vi "Copy.vi"(8 "error in":errorcluster, 9 "Target Folder":path, 10 "Source":path, 11 "File Manager in":refnum<class "File Manager.lvclass">) -> (0 "error out":errorcluster, 2 "New Path":path, 3 "File Manager out":refnum<class "File Manager.lvclass">)   [LabVIEW 2026, in "File Manager.lvclass"]
doc: "This VI copies the specified source to the target directory. If the target already exists it will be overwritten."
uses:
  File Manager.lvclass
  File Manager.lvclass/File Manager.ctl
  Interfaces/ILogger/ILogger Messages/Log Msg/Log Msg.lvclass/Log Msg.ctl
  <vilib>/ActorFramework/Message Enqueuer/Message Enqueuer.lvclass/Message Enqueuer.ctl
  <vilib>/ActorFramework/Message Enqueuer/Enqueue.vi
  Interfaces/ILogger/ILogger Messages/Log Msg/Log Msg.lvclass
  <userlib>/_OpenG.lib/file/file.llb/Strip Path Extension - Path__ogtk.vi
  <vilib>/ActorFramework/Message Priority Queue/Priority Enqueue.vi
  <userlib>/_OpenG.lib/file/file.llb/openg_file.lvlib
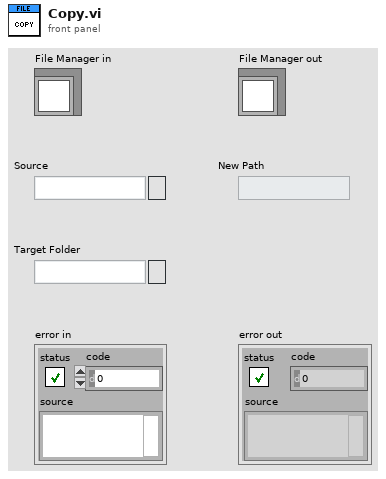
[diagram p1: front panel]
types:
  T1 = typedef "Log Entry--cluster.ctl" = cluster{"Time":timestamp, "Message":string}
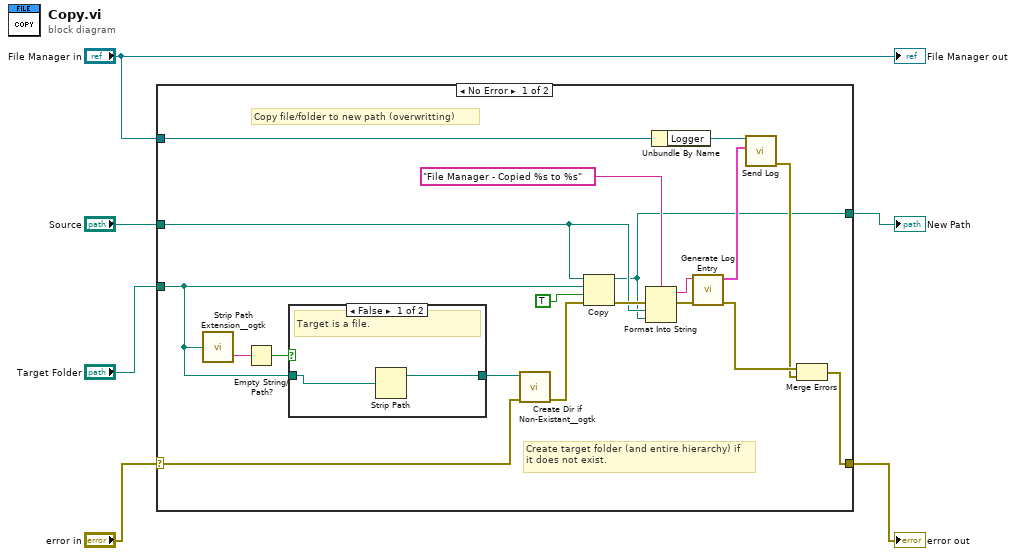
[diagram p0: block diagram]
diagram:
  n1 = case shown="No Error" "error in" {
    selector: "error in" -> [w8 w29]
    tunnel: [w25 w29] -> w6
    tunnel: "File Manager in" -> [w20 _]
    tunnel: "Source" -> [w14 _]
    tunnel: [w13 _] -> w2
    tunnel: "Target Folder" -> [w10 _]
    frame No Error {
      # "Create target folder (and entire hierarchy) if\nit does not exist."
      # "Copy file/folder to new path (overwritting)"
      n2 = call-poly <userlib>:"Strip Path Extension__ogtk.vi"("path"=w10) -> ("extension"=w12:string)  [unwired: 1 out]
      n3 = Empty String/Path?(string/path=w12) -> (empty?=w11:bool)
      n4 = case shown="False" w11 {
        tunnel: w10 -> [w27 w28]
        tunnel: [w26 w28] -> w9
        frame False {
          # "Target is a file."
          n5 = Strip Path(path=w27) -> (stripped path=w26:path)  [unwired: 1 out]
        }
        frame True {
          # "Target is a folder"
        }
      }
      n6 = call <userlib>:"Create Dir if Non-Existant__ogtk.vi"("error in (no error)"=w8, "Directory Path"=w9) -> ("error out"=w7:errorcluster)  [unwired: 7 in, 2 out]
      n7 = Copy(8:w7, 9:TRUE ("overwrite (F)"), 10:w10, 11:w14) -> (0:w21:errorcluster, 3:w13:path)  [unwired: 1 in, 1 out]
      n8 = Format Into String(format string="File Manager - Copied %s to %s" ("Message"), error in=w21, w14, w13) -> (resulting string=w16:string, error out=w23:errorcluster)  [unwired: 1 in]
      n9 = Unbundle By Name(w20) -> ("Logger"=w19:refnum<class "Message Enqueuer.lvclass">)
      n10 = call "Generate Log Entry.vi"("error in"=w23, "Message"=w16) -> ("error out"=w24:errorcluster, "Log Entry"=w18:T1)  [unwired: 8 in]
      n11 = call "Send Log.vi"("Log Entry"=w18, "Message Enqueuer"=w19) -> ("error out"=w22:errorcluster)  [unwired: 8 in, 1 out]
      n12 = Merge Errors(w24, w22) -> (w25:errorcluster)
    }
    frame Error {
      # "Pass error without further actions."
    }
  }
  "error out" <- w6
  "New Path" <- w2
  "File Manager out" <- "File Manager in"
